vi "Room_Blit.vi"(0 "Picture":u8[][](array[numeric]), 1 "FloorPhase":i32, 2 "View":T1={"Hide"=FALSE, "CX"=0, "CY"=0, "ClaudeIdx"=-1, "ClaudeX"=0, "ClaudeY"=0}, 5 "Sprites":cluster{"Pix":u8[][], "Mask":u8[][]}[](array[cluster]), 7 "Tiles":u8[][](array[numeric]), 9 "Region":T2={"left"=0, "top"=0, "right"=40, "bottom"=20}, 11 "error in":errorcluster) -> (4 "Picture out":u8[][](array[numeric]), 15 "error out":errorcluster)   [LabVIEW 2020, in "GH_Render.lvlib"]
doc: "Draws the objects of a room inside Region (tiles; two rows more upwards for the doors): vanishing floors (FloorPhase 0 normal, 1 warning, 2 gone), conveyors, doors (only at their top tile), keys, gold and the torch. Hide = dark room: only objects within the light (distance^2 <= 28 tiles from CX, CY) are drawn."
uses:
  GH_Render.lvlib
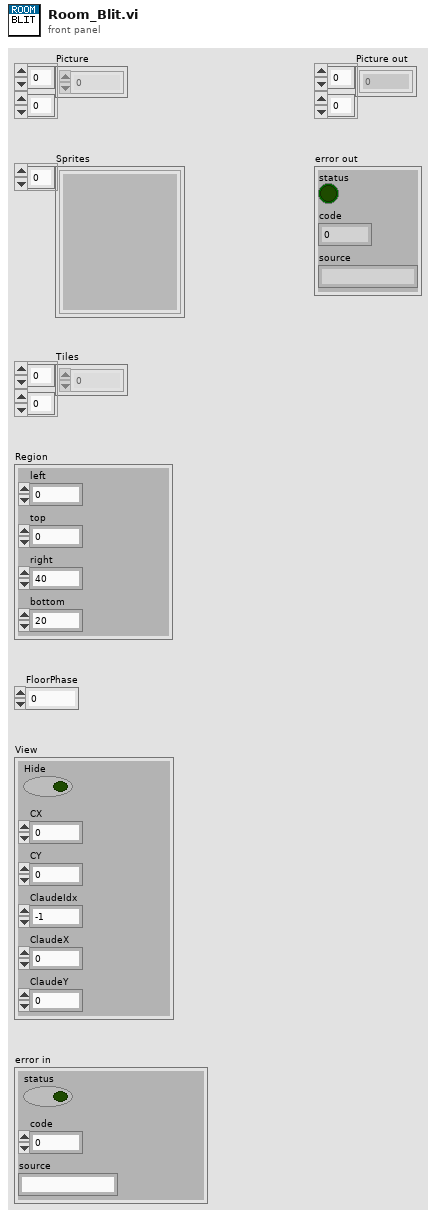
[diagram p1: front panel]
types:
  T1 = cluster{"Hide":bool, "CX":i32, "CY":i32, "ClaudeIdx":i32, "ClaudeX":i32, "ClaudeY":i32}
  T2 = cluster{"left":i16, "top":i16, "right":i16, "bottom":i16}
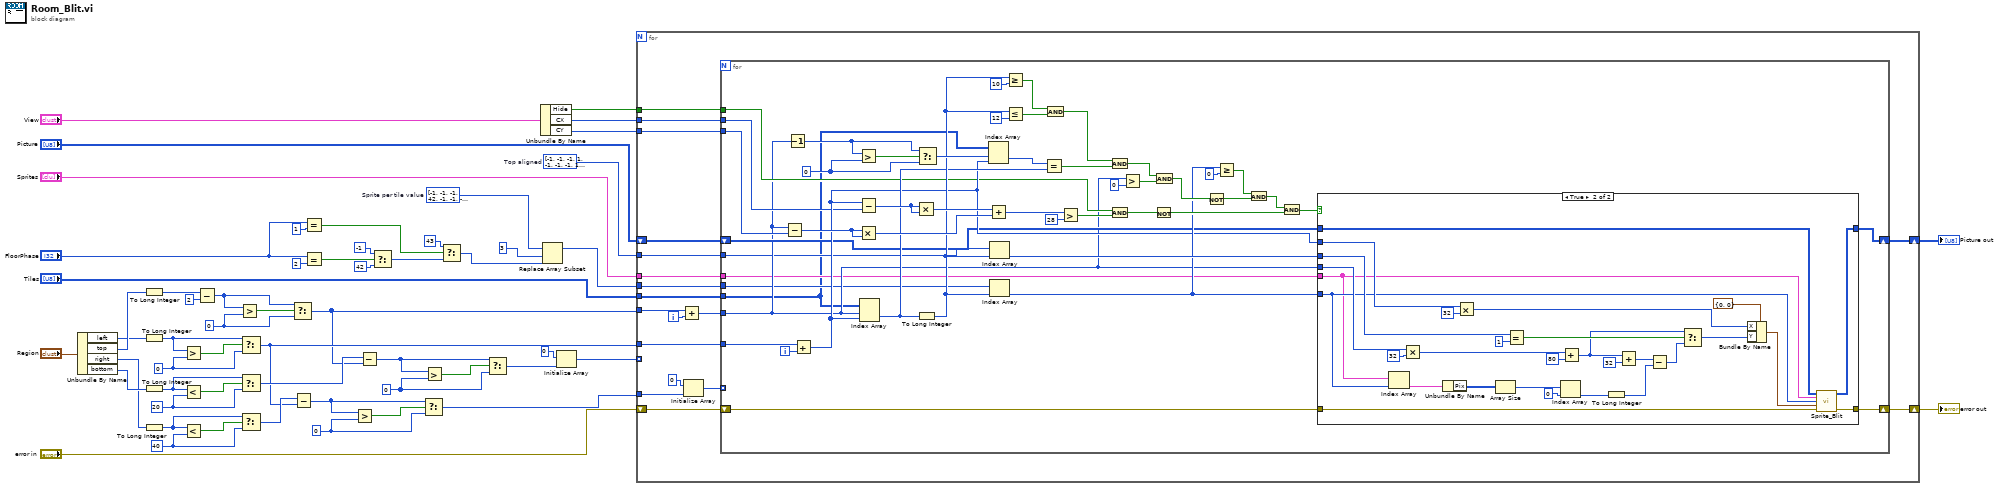
[diagram p0: block diagram]
diagram:
  w37 = 0
  w33 = 40
  w30 = 0
  w26 = 20
  w23 = 0
  w20 = 0
  w9 = i32[] [-1, -1, -1, 1, -1, -1, -1, 1, 1, -1, 1, 1, 1, -1, -1, -1, -1, -1, -1, -1, -1, -1, -1]  # Top aligned
  w8 = i32[] [-1, -1, -1, 42, -1, -1, -1, 48, 44, -1, 37, 38, 39, 34, 35, 36, 28, 32, 40, -1, -1, -1, -1]  # Sprite per tile value
  n1 = Unbundle By Name("Region") -> ("left"=w10:i16, "top"=w11:i16, "right"=w12:i16, "bottom"=w13:i16)
  n2 = To Long Integer(number=w11) -> (32bit integer=w15:i32)
  n3 = To Long Integer(number=w10) -> (32bit integer=w14:i32)
  n4 = To Long Integer(number=w13) -> (32bit integer=w17:i32)
  n5 = To Long Integer(number=w12) -> (32bit integer=w16:i32)
  n6 = Greater?(x=w14, y=w23) -> (0:w24:bool)
  n7 = Less?(x=w17, y=w26) -> (x < y?=w27:bool)
  n8 = Less?(x=w16, y=w33) -> (x < y?=w34:bool)
  n9 = Subtract(x=w15, y=2) -> (x-y=w19:i32)
  n10 = Greater?(x=w19, y=w20) -> (0:w21:bool)
  n11 = Select(t=w14, s=w24, f=w23) -> (s? t:f=w25:i32)
  n12 = Select(t=w17, s=w27, f=w26) -> (s? t:f=w28:i32)
  n13 = Select(t=w16, s=w34, f=w33) -> (s? t:f=w35:i32)
  n14 = Select(t=w19, s=w21, f=w20) -> (s? t:f=w22:i32)
  n15 = Subtract(x=w35, y=w25) -> (x-y=w36:i32)
  n16 = Equal?(x="FloorPhase", y=1) -> (x = y?=w44:bool)
  n17 = Equal?(x="FloorPhase", y=2) -> (x = y?=w47:bool)
  n18 = Greater?(x=w36, y=w37) -> (0:w38:bool)
  n19 = Subtract(x=w28, y=w22) -> (x-y=w29:i32)
  n20 = Select(t=-1, s=w47, f=42) -> (s? t:f=w50:i32)
  n21 = Select(t=w36, s=w38, f=w37) -> (s? t:f=w39:i32)
  n22 = Greater?(x=w29, y=w30) -> (0:w31:bool)
  n23 = Select(t=43, s=w44, f=w50) -> (s? t:f=w51:i32)
  n24 = Select(t=w29, s=w31, f=w30) -> (s? t:f=w32:i32)
  n25 = Unbundle By Name("View") -> ("Hide"=w40:bool, "CX"=w41:i32, "CY"=w42:i32)
  n26 = Replace Array Subset(array=w8, new element=w51, index=3) -> (w53:i32[])
  n27 = Initialize Array(0, w32) -> (w55:i32[])
  n28 = for {
    tunnel: "Tiles" -> [w59]
    tunnel: "Sprites" -> [w60]
    tunnel: w9 -> [w62]
    shift-right: [w70] -> w56
    shift-left: "Picture" -> [w69]
    shift-right: [w72] -> w57
    shift-left: "error in" -> [w71]
    tunnel: w40 -> [w66]
    tunnel: w41 -> [w67]
    tunnel: w42 -> [w68]
    tunnel: w53 -> [w61]
    tunnel: w25 -> [w64]
    tunnel: w22 -> [w63]
    tunnel: w39 -> [w65]
    tunnel: w55 -> [_] mode=indexing
    i -> [w58]
    n29 = Add(x=w63, y=w58) -> (x+y=w73:i32)
    n30 = Initialize Array(0, w65) -> (w75:i32[])
    n31 = for {
      tunnel: w59 -> [w77]
      tunnel: w60 -> [w78]
      tunnel: w62 -> [w80]
      shift-right: [w87] -> w70
      shift-left: w69 -> [w86]
      shift-right: [w89] -> w72
      shift-left: w71 -> [w88]
      tunnel: w66 -> [w83]
      tunnel: w67 -> [w84]
      tunnel: w68 -> [w85]
      tunnel: w61 -> [w79]
      tunnel: w64 -> [w82]
      tunnel: w73 -> [w81]
      tunnel: w75 -> [_] mode=indexing
      i -> [w76]
      w95 = 0
      n32 = Subtract(x=w81, y=w85) -> (x-y=w110:i32)
      n33 = Decrement(x=w81) -> (x-1=w94:i32)
      n34 = Add(x=w82, y=w76) -> (x+y=w90:i32)
      n35 = Greater?(x=w94, y=w95) -> (0:w96:bool)
      n36 = Multiply(x=w110, y=w110) -> (x*y=w112:i32)
      n37 = Subtract(x=w90, y=w84) -> (x-y=w109:i32)
      n38 = Index Array(array=w77, index (row)=w81, index (col)=w90) -> (element=w91:u8)
      n39 = Multiply(x=w109, y=w109) -> (x*y=w111:i32)
      n40 = To Long Integer(number=w91) -> (32bit integer=w92:i32)
      n41 = Select(t=w94, s=w96, f=w95) -> (s? t:f=w97:i32)
      n42 = Index Array(array=w77, index (row)=w97, index (col)=w90) -> (element=w98:u8)
      n43 = Add(x=w111, y=w112) -> (x+y=w113:i32)
      n44 = Index Array(array=w80, index=w92) -> (element=w123:i32)
      n45 = Index Array(array=w79, index=w92) -> (element=w93:i32)
      n46 = Greater Or Equal?(x=w92, y=10) -> (x >= y?=w100:bool)
      n47 = Less Or Equal?(x=w92, y=12) -> (x <= y?=w102:bool)
      n48 = Equal?(x=w98, y=w91) -> (x = y?=w104:bool)
      n49 = And(x=w100, y=w102) -> (x .and. y?=w103:bool)
      n50 = Greater?(x=w113, y=28) -> (0:w115:bool)
      n51 = And(x=w103, y=w104) -> (x .and. y?=w107:bool)
      n52 = And(x=w83, y=w115) -> (x .and. y?=w116:bool)
      n53 = Greater?(x=w81, y=0) -> (0:w106:bool)
      n54 = Not(x=w116) -> (.not. x?=w120:bool)
      n55 = And(x=w107, y=w106) -> (x .and. y?=w108:bool)
      n56 = Not(x=w108) -> (.not. x?=w119:bool)
      n57 = Greater Or Equal?(x=w93, y=0) -> (x >= y?=w118:bool)
      n58 = And(x=w118, y=w119) -> (x .and. y?=w121:bool)
      n59 = And(x=w121, y=w120) -> (x .and. y?=w122:bool)
      n60 = case shown="True" w122 {
        tunnel: w86 -> [w124 w126]
        tunnel: w78 -> [_ w127]
        tunnel: w88 -> [w125 w129]
        tunnel: w90 -> [_ w131]
        tunnel: w81 -> [_ w130]
        tunnel: w93 -> [_ w128]
        tunnel: w123 -> [_ w132]
        tunnel: [w124 w153] -> w87
        tunnel: [w125 w154] -> w89
        frame False {
        }
        frame True {
          n61 = Index Array(array=w127, index=w128) -> (element=w133:cluster{"Pix":u8[][], "Mask":u8[][]})
          n62 = Multiply(x=w130, y=32) -> (x*y=w140:i32)
          n63 = Unbundle By Name(w133) -> ("Pix"=w134:u8[][])
          n64 = Multiply(x=w131, y=32) -> (x*y=w151:i32)
          n65 = Array Size(array=w134) -> (size(s)=w135:i32[])
          n66 = Equal?(x=w132, y=1) -> (x = y?=w144:bool)
          n67 = Index Array(array=w135, index=0) -> (element=w137:i32)
          n68 = Add(x=w140, y=80) -> (x+y=w142:i32)
          n69 = To Long Integer(number=w137) -> (32bit integer=w138:i32)
          n70 = Add(x=w142, y=32) -> (x+y=w146:i32)
          n71 = Subtract(x=w146, y=w138) -> (x-y=w147:i32)
          n72 = Select(t=w142, s=w144, f=w147) -> (s? t:f=w148:i32)
          n73 = Bundle By Name(cluster=cluster{"X":i32, "Y":i32} {"X"=0, "Y"=0}, "X"=w151, "Y"=w148) -> (w152:cluster{"X":i32, "Y":i32})
          n74 = call "Sprite_Blit.vi"("Picture"=w126, "Sprites"=w127, "Index"=w128, "Position"=w152, "error in"=w129) -> ("Picture out"=w153:u8[][], "error out"=w154:errorcluster)  [unwired: 9 in]
        }
      }
    }
  }
  "Picture out" <- w56
  "error out" <- w57
